vi "Registry_Update.vi"(8 "error in (no error)":errorcluster={"status"=FALSE, "code"=0, "source"="\"\""}, 10 "typed value":string, 11 "Parameter ID":string) -> (0 "error out":errorcluster={"status"=FALSE, "code"=0, "source"="\"\""}, 2 "status ok":bool, 3 "Registry update result":string)   [LabVIEW 2026]
doc: "INTENT: Publish producer data. LOGIC: Check producer identity, expected type and monotonic sample sequencing; overwrite latest value atomically in registry owner."
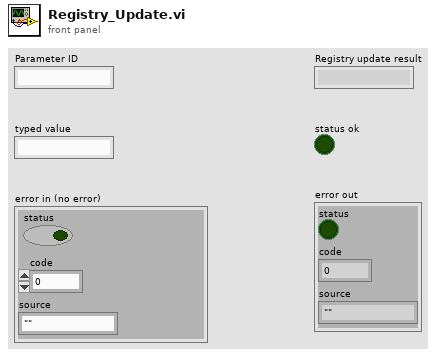
[diagram p1: front panel]
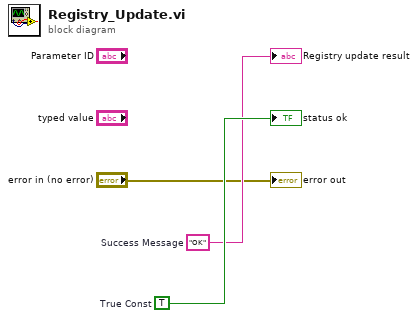
[diagram p0: block diagram]
diagram:
  w3 = TRUE  # True Const
  w2 = "OK"  # Success Message
  "Registry update result" <- w2
  "status ok" <- w3
  "error out" <- "error in (no error)"
